vi "uService GUI.vi"(8 "error in (no error)":errorcluster, 11 "uService Template in":refnum<class "Scheduler.lvclass">) -> (3 "uService Template out":refnum<class "Scheduler.lvclass">)   [LabVIEW 2020, in "Scheduler.lvlib" / "Scheduler.lvclass"]
uses:
  Scheduler.lvclass
  C:/LabVIEW Code/CIRCUS/TALOS/TALOS_PPL.lvlibp/Father of all uServices/Father of all uServices/Father of all uServices.lvclass
  Run Utilities/Sequence of SBlocks/Sequence of SBlcoks - GUI.ctl
  Run Utilities/Schedule Block/Schedule Block - simplified GUI.ctl
  Run Utilities/TypeDefs/Synchronize FPGA Cluster.ctl
  Append Options.ctl
  Scheduler Consumer Case Selector.ctl
  Selection.ctl
  TALOS/TALOS_PPL.lvlibp/Father of all uServices/Father of all uServices/Father of all uServices.lvclass
  Scheduler.lvclass/Scheduler.ctl
  C:/LabVIEW Code/CIRCUS/TALOS/TALOS_PPL.lvlibp/Ancestor/Ancestor/Ancestor.lvclass
  C:/LabVIEW Code/CIRCUS/TALOS/Actor Framework.lvlibp/1abvi3w/vi.lib/ActorFramework/Actor/Actor.lvclass
  C:/LabVIEW Code/CIRCUS/CIRCUS uServices et al/Scheduler/Scheduler.lvclass
  Run Utilities/Sequence of SBlocks/Sequence of SBlocks.lvclass
  Run Utilities/Run Utilities.lvlib
  Run Utilities/Schedule Block/Schedule Block.lvclass
panel:
  in  "Append":T1
  in  "SB Buttons":T2
  in  "Add RUN":bool
  out "Sync. mask":T3[](array[typedef])
  in  "Parallel":bool
  in  "Reload parameters":bool
  in  "Array of Sequences":T4[](array[typedef])
  in  "Science":bool
  in  "Save":bool
  in  "Load":bool
  in  "Reset":bool
  in  "stop Scheduler":bool
  # "SCHEDULER"
  # "Schedule block manipulation"
  # "Multi FPGA Operation"
  # "Sync. mask"
  # "Estimated time of execution"
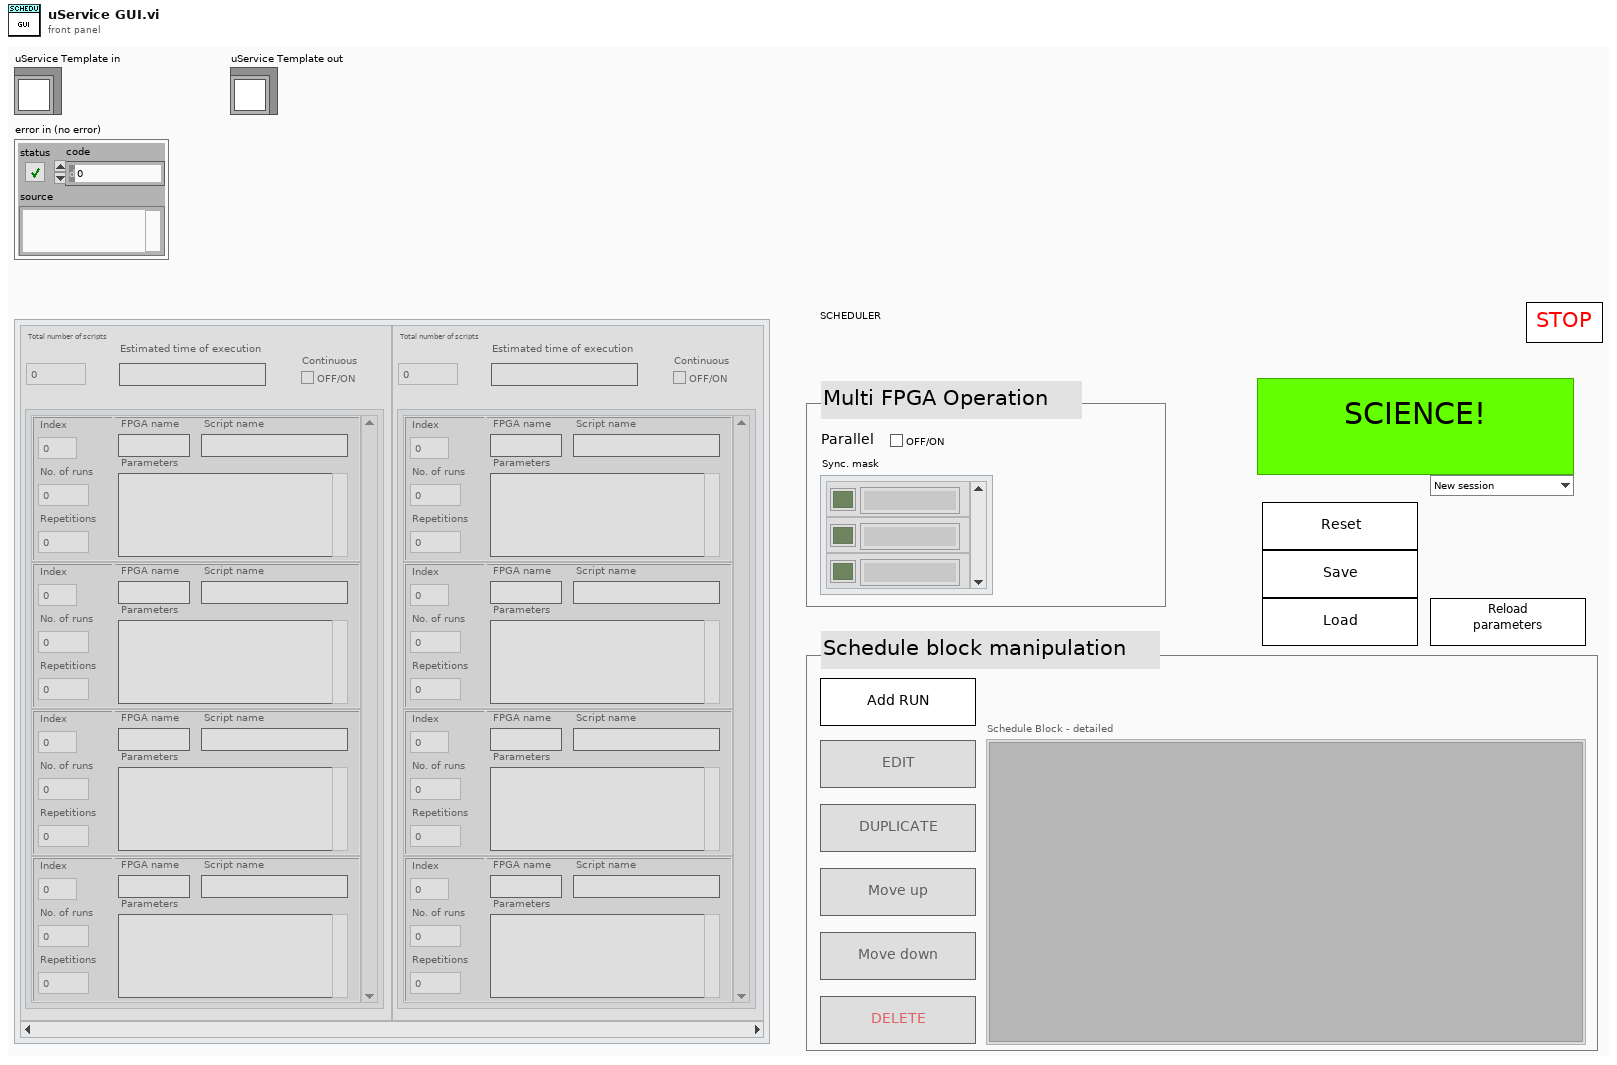
[diagram p1: front panel]
types:
  T1 = typedef "Scheduler.lvlib/Scheduler.lvclass/Append Options.ctl" = enum16{"New session", "Append to bottom", "Append to top"}
  T2 = cluster{"Move up SB":bool, "Move down SB":bool, "DELETE_SB":bool, "DUPLICATE_SB":bool, "EDIT_SB":bool}
  T3 = typedef "Run Utilities.lvlib/Synchronize FPGA Cluster.ctl" = cluster{"Status":bool, "FPGA Name":string}
  T4 = typedef "Run Utilities.lvlib/Sequence of SBlocks.lvclass/Sequence of SBlcoks - GUI.ctl" = cluster{"Total number of scripts":i32, "Time":string, "Sequence of SBlocks":T5[], "Continuous":bool}
  T5 = typedef "Run Utilities.lvlib/Schedule Block.lvclass/Schedule Block - simplified GUI.ctl" = cluster{"Bcg Color":u32, "Index":i32, "No. of runs":i32, "Script name":string, "FPGA name":string, "Parameters":string, "Repetitions":i32}
  T6 = enum16{"New session", "Append to bottom", "Append to top"}
  T7 = typedef "Scheduler.lvlib/Scheduler.lvclass/Scheduler Consumer Case Selector.ctl" = enum16{"Add SBlock", "Update GUI", "Move SBlock", "Select SBlock", "Update Cont.", "Load", "Save", "Reset", "Send to Tamer", "Edit SBlock", "Duplicate SBlock", "Delete SBlock", "Update SBlock", "Init", "Split/Combine Schedules", "Reschedule", "Load Parameters"}
  T8 = typedef "Scheduler.lvlib/Scheduler.lvclass/Selection.ctl" = cluster{"Row":i32, "Column":i32}
  T9 = typedef "TALOS.lvlib/Run Utilities.lvlib/Synchronize Kasli Cluster.ctl" = cluster{"Status":bool, "FPGA Name":string}
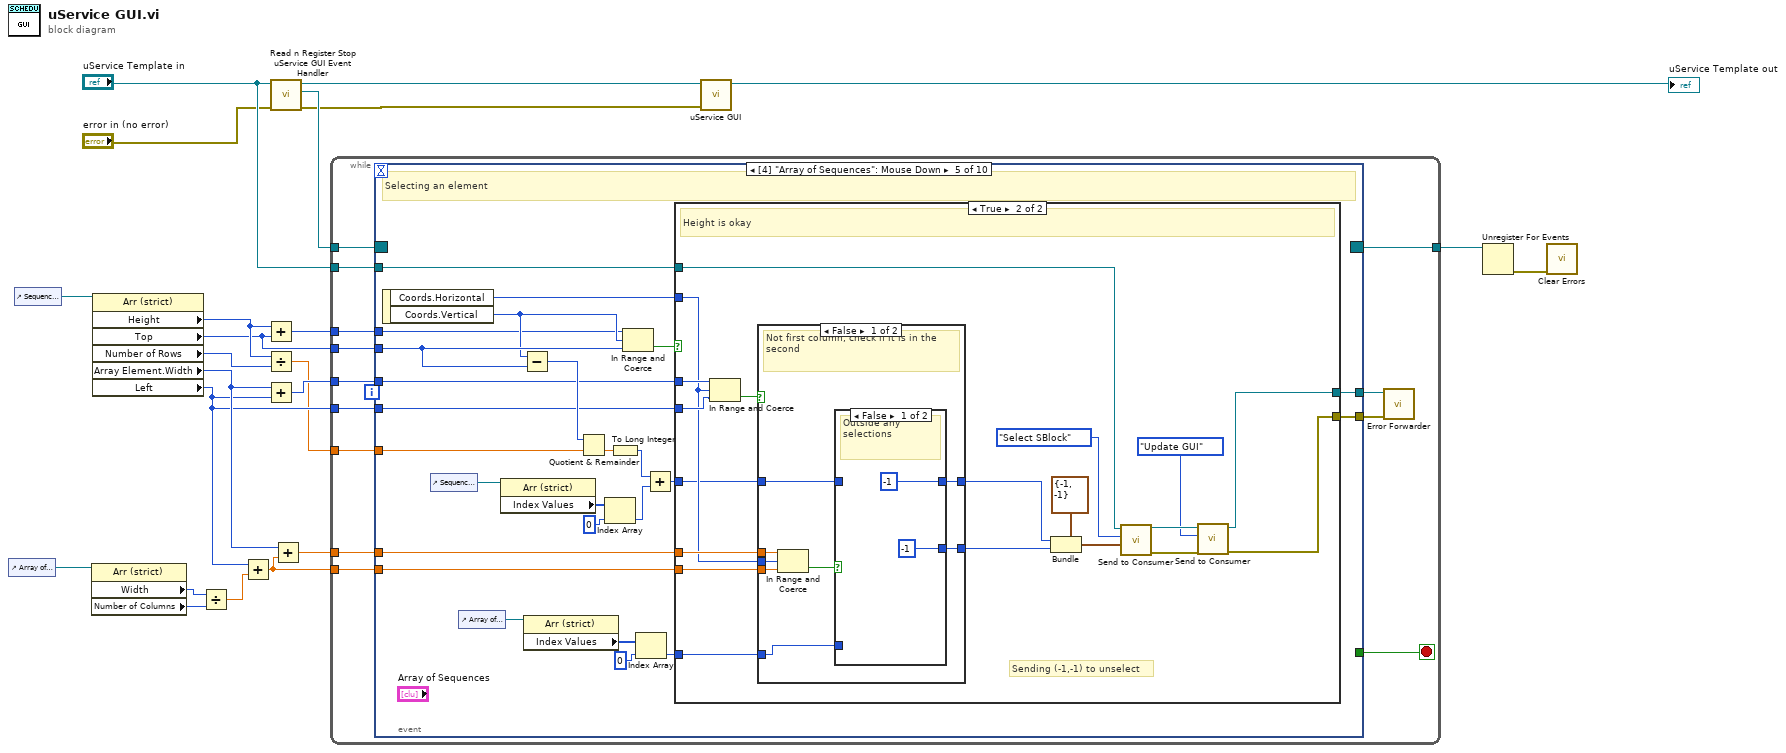
[diagram p0: block diagram]
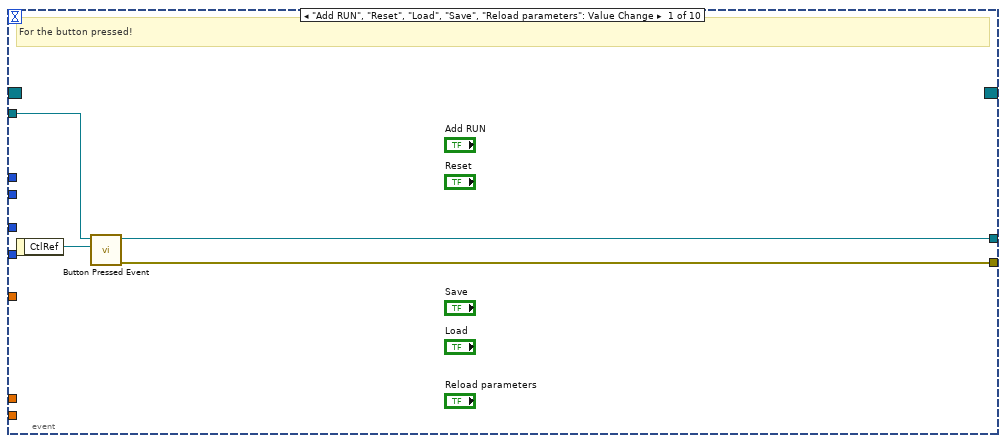
[diagram p2: hidden frame]
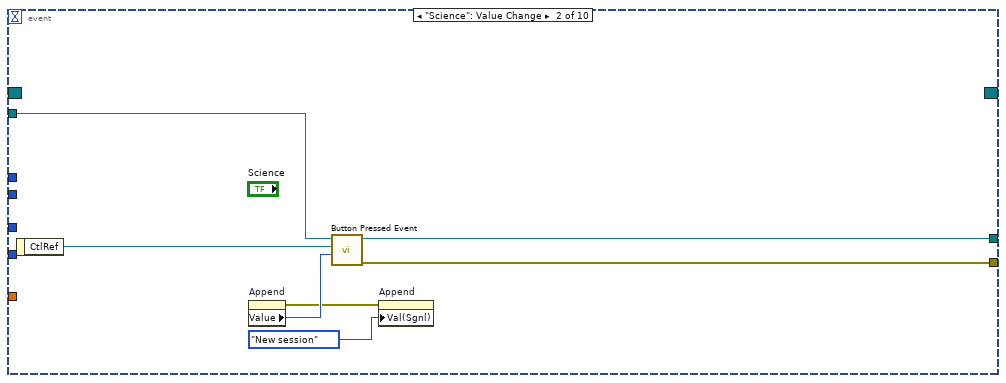
[diagram p3: hidden frame]
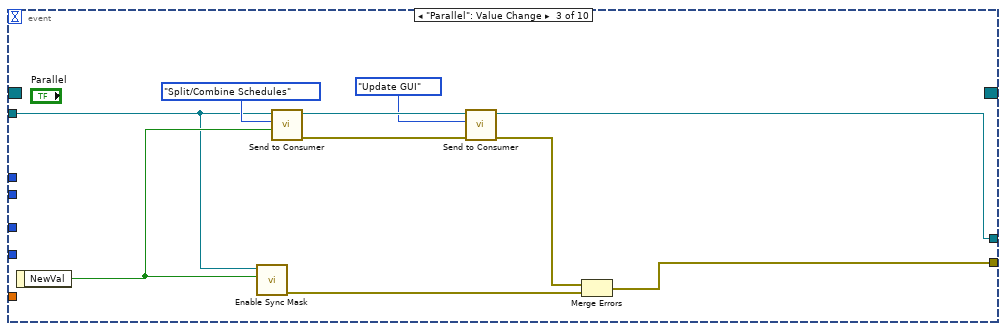
[diagram p4: hidden frame]
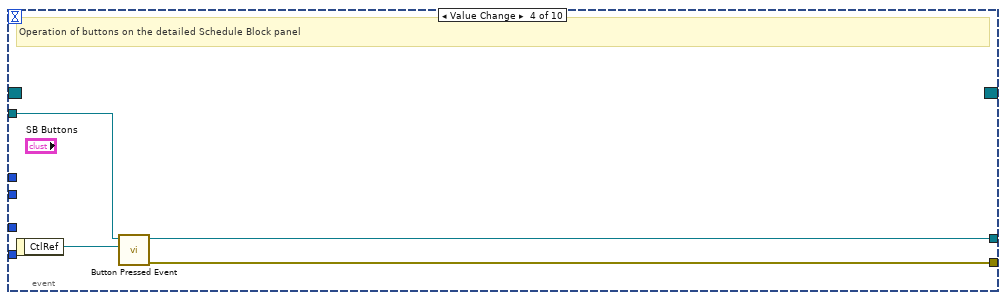
[diagram p5: hidden frame]
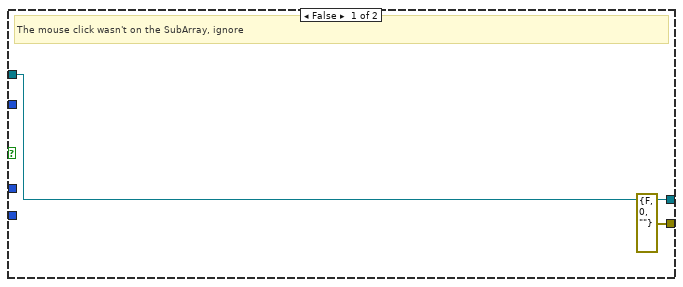
[diagram p6: hidden frame]
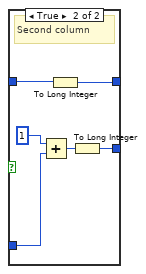
[diagram p7: hidden frame]
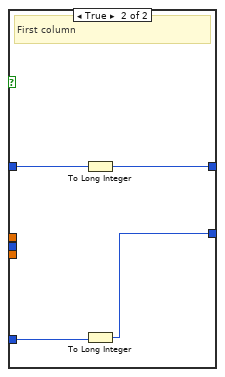
[diagram p8: hidden frame]
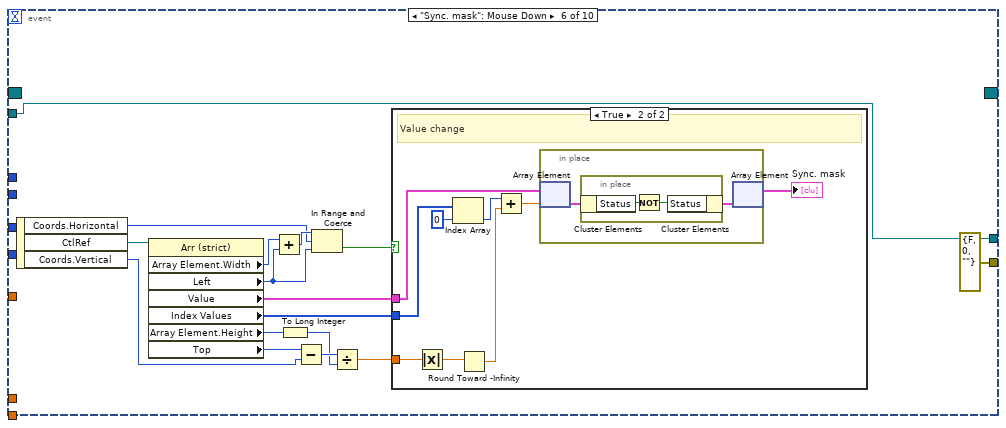
[diagram p9: hidden frame]
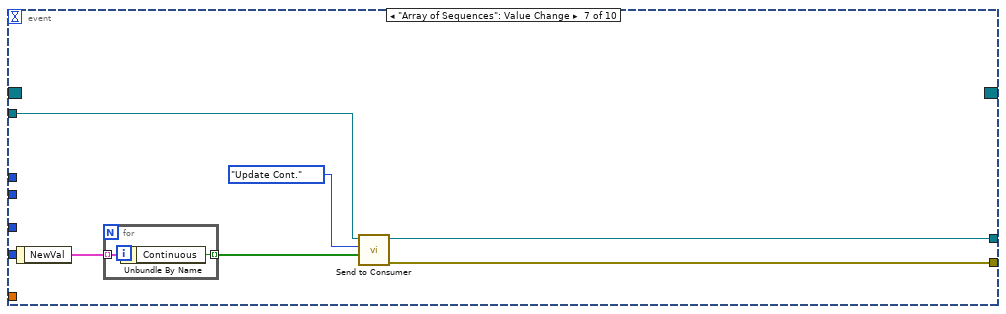
[diagram p11: hidden frame]
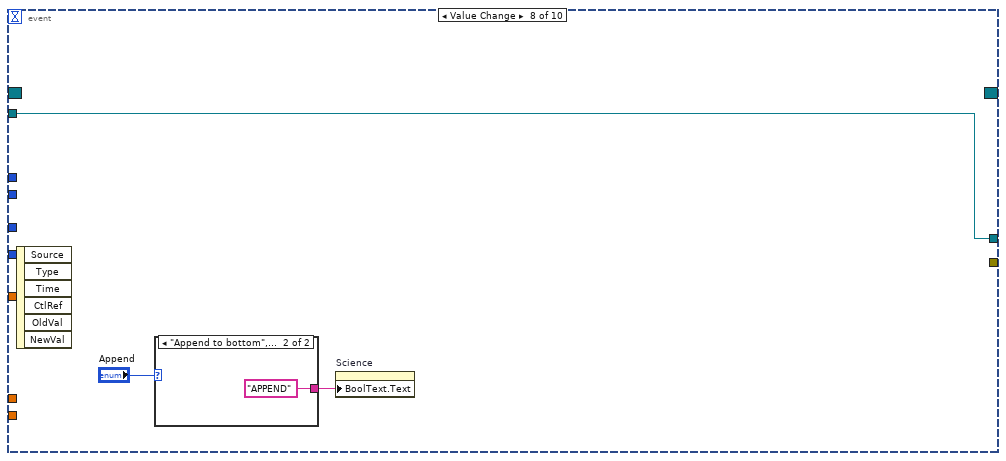
[diagram p12: hidden frame]
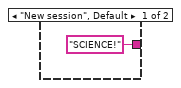
[diagram p13: hidden frame]
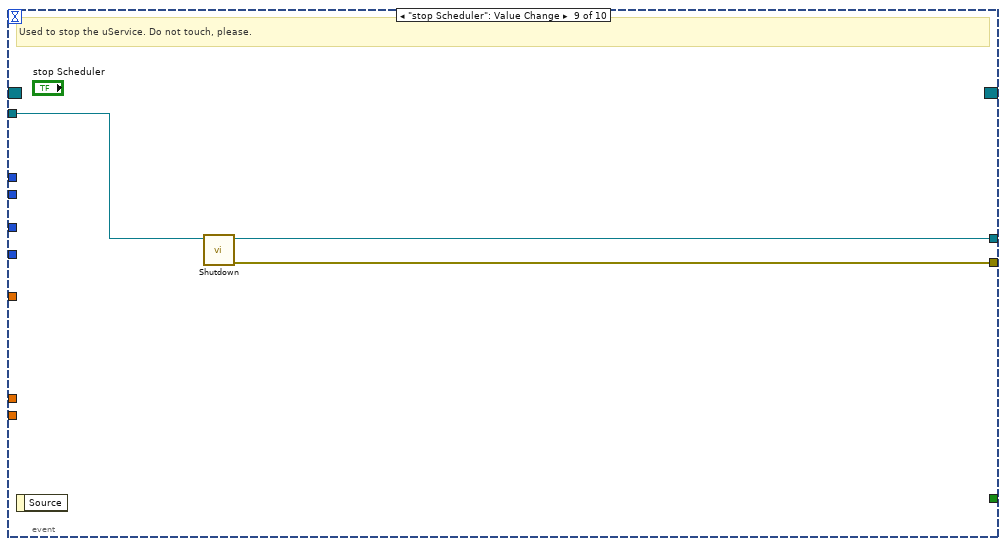
[diagram p14: hidden frame]
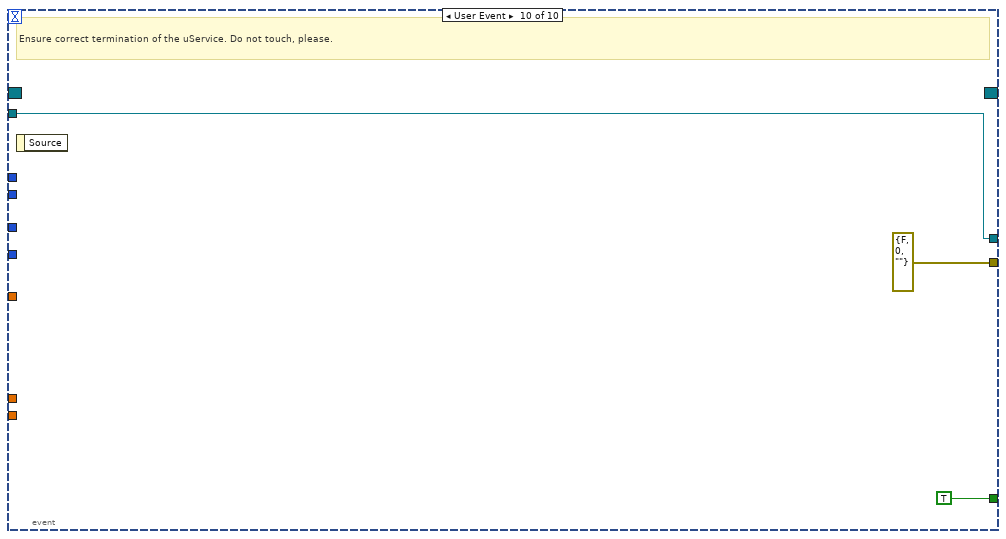
[diagram p15: hidden frame]
diagram:
  n1 = control-ref of="Array of Sequences"() -> (w5:refnum<vi>)
  n2 = control-ref of="Sequence of SBlocks"() -> (w4:refnum<vi>)
  n3 = property class="Arr (strict)"(reference=w5) -> ("Width"=w17:u32, "Number of Columns"=w2:u32)  [unwired: 1 in, 2 out]
  n4 = property class="Arr (strict)"(reference=w4) -> ("Height"=w16:u32, "Top"=w11:i32, "Number of Rows"=w15:u32, "Array Element.Width"=w13:u32, "Left"=w9:i32)  [unwired: 1 in, 2 out]
  n5 = Divide(x=w17, y=w2) -> (x/y=w14:dbl)
  n6 = Add(x=w9, y=w14) -> (x+y=w6:dbl)
  n7 = Add(x=w16, y=w11) -> (x+y=w12:u32)
  n8 = Divide(x=w16, y=w15) -> (x/y=w8:dbl)
  n9 = Add(x=w13, y=w9) -> (x+y=w10:u32)
  n10 = call-dynamic "Read n Register Stop uService GUI Event Handler .vi"("error in (no error)"="error in (no error)", "uService Template in"="uService Template in") -> ("error out"=w3:errorcluster, "Stop uService GUI Event Ref"=w18:refnum<event-registration>, "uService Template out"=w19:refnum<class "Scheduler.lvclass">)  [unwired: 7 in]
  n11 = Add(x=w13, y=w6) -> (x+y=w7:dbl)
  n12 = while {
    tunnel: [w36] -> w20
    tunnel: w18 -> [w34]
    tunnel: "uService Template in" -> [w33]
    tunnel: w12 -> [w32]
    tunnel: w11 -> [w31]
    tunnel: w10 -> [w30]
    tunnel: w9 -> [w29]
    tunnel: w8 -> [w28]
    tunnel: w7 -> [w27]
    tunnel: w6 -> [w26]
    stop <- w35 stop-if-true
    n13 = event shown="[4] \"Array of Sequences\": Mouse Down" {
      selector: w34 -> [_ _ _ _ _ _ _ _ _ _]
      dyn-events: [_ _ _ _ _ _ _ _ _ _] -> w36
      timeout: _ -> [_ _ _ _ _ _ _ _ _ _]
      tunnel: [_ _ _ _ _ _ _ _ _ TRUE] -> w35
      tunnel: w33 -> [w40 w47 w52 w60 w68 w129 w161 w167 w172 w174]
      tunnel: w32 -> [_ _ _ _ w64 _ _ _ _ _]
      tunnel: w31 -> [_ _ _ _ w75 _ _ _ _ _]
      tunnel: w30 -> [_ _ _ _ w74 _ _ _ _ _]
      tunnel: w29 -> [_ _ _ _ w73 _ _ _ _ _]
      tunnel: w28 -> [_ _ _ _ w72 _ _ _ _ _]
      tunnel: w27 -> [_ _ _ _ w71 _ _ _ _ _]
      tunnel: w26 -> [_ _ _ _ w65 _ _ _ _ _]
      tunnel: [w38 w46 w48 w59 w63 w129 w158 w167 w171 w174] -> w25
      tunnel: [w37 w45 w49 w58 w62 errorcluster {"status"=FALSE, "code"=0, "source"=""} ("error out") w157 _ w170 errorcluster {"status"=FALSE, "code"=0, "source"=""} ("error out")] -> w24
      event "Add RUN", "Reset", "Load", "Save", "Reload parameters": Value Change {
        # "For the button pressed!"
        n14 = event-data() -> ("CtlRef"=w39:refnum<vi>)  [unwired: 1 in]
        n15 = call-dynamic "Button Pressed Event.vi"("CtlRef"=w39, "uService Template in"=w40) -> ("error out"=w37:errorcluster, "uService Template out"=w38:refnum<class "Scheduler.lvclass">)  [unwired: 8 in]
      }
      event "Science": Value Change {
        n16 = event-data() -> ("CtlRef"=w44:refnum<vi>)  [unwired: 1 in]
        n17 = property on="Append" class="Enum (strict)"() -> (error out=w41:errorcluster, "Value"=w43:T1)  [unwired: 2 in, 1 out]
        n18 = call-dynamic "Button Pressed Event.vi"("Data"=w43, "CtlRef"=w44, "uService Template in"=w47) -> ("error out"=w45:errorcluster, "uService Template out"=w46:refnum<class "Scheduler.lvclass">)  [unwired: 7 in]
        n19 = property on="Append" class="Enum (strict)"(error in=w41, "Val(Sgnl)"=T6."New session" ("Append")) -> ()  [unwired: 1 in, 2 out]
      }
      event "Parallel": Value Change {
        n20 = event-data() -> ("NewVal"=w53:bool)  [unwired: 1 in]
        n21 = call-dynamic "Enable Sync Mask.vi"("Enable"=w53, "Scheduler in"=w52) -> ("error out"=w50:errorcluster)  [unwired: 8 in, 1 out]
        n22 = call "Send to Consumer.vi"("Data"=w53, "Case ID"=Scheduler_Consumer_Case_Selector."Split/Combine Schedules" ("Shifter Panel Consumer Case Selector"), "uService Template in"=w52) -> ("error out"=w54:errorcluster, "uService Template out"=w57:refnum<class "Scheduler.lvclass">)  [unwired: 7 in]
        n23 = call "Send to Consumer.vi"("error in (no error)"=w54, "Case ID"=Scheduler_Consumer_Case_Selector."Update GUI" ("Shifter Panel Consumer Case Selector"), "uService Template in"=w57) -> ("error out"=w51:errorcluster, "uService Template out"=w48:refnum<class "Scheduler.lvclass">)  [unwired: 7 in]
        n24 = Merge Errors(w51, w50) -> (w49:errorcluster)
      }
      event "SB Buttons.Move up SB", "SB Buttons.Move down SB", "SB Buttons.DELETE_SB", "SB Buttons.DUPLICATE_SB", "SB Buttons.EDIT_SB": Value Change {
        # "Operation of buttons on the detailed Schedule Block panel"
        n25 = event-data() -> ("CtlRef"=w61:refnum<vi>)  [unwired: 1 in]
        n26 = call-dynamic "Button Pressed Event.vi"("CtlRef"=w61, "uService Template in"=w60) -> ("error out"=w58:errorcluster, "uService Template out"=w59:refnum<class "Scheduler.lvclass">)  [unwired: 8 in]
      }
      event "Array of Sequences": Mouse Down {
        # "Selecting an element"
        n27 = event-data() -> ("Coords.Horizontal"=w70:i32, "Coords.Vertical"=w69:i32)  [unwired: 1 in]
        n28 = control-ref of="Sequence of SBlocks"() -> (w67:refnum<vi>)
        n29 = control-ref of="Array of Sequences"() -> (w66:refnum<vi>)
        n30 = property class="Arr (strict)"(reference=w67) -> ("Index Values"=w80:u32[])  [unwired: 1 in, 2 out]
        n31 = Subtract(x=w69, y=w75) -> (x-y=w82:i32)
        n32 = property class="Arr (strict)"(reference=w66) -> ("Index Values"=w85:u32[])  [unwired: 1 in, 2 out]
        n33 = Quotient & Remainder(x=w82, y=w72) -> (floor(x/y)=w81:dbl)  [unwired: 1 out]
        n34 = Index Array(array=w80, index=0) -> (element=w77:u32)
        n35 = To Long Integer(number=w81) -> (32bit integer=w79:i32)
        n36 = In Range and Coerce(upper limit=w64, x=w69, lower limit=w75) -> (In Range?=w86:bool)  [unwired: 1 out]
        n37 = Index Array(array=w85, index=0) -> (element=w83:u32)
        n38 = Add(x=w79, y=w77) -> (x+y=w76:u32)
        n39 = case shown="True" w86 {
          tunnel: w74 -> [_ w107]
          tunnel: w73 -> [_ w106]
          tunnel: w70 -> [_ w102]
          tunnel: w71 -> [_ w104]
          tunnel: w65 -> [_ w103]
          tunnel: w83 -> [_ w101]
          tunnel: w76 -> [_ w100]
          tunnel: w68 -> [w88 w99]
          tunnel: [w88 w89] -> w63
          tunnel: [errorcluster {"status"=FALSE, "code"=0, "source"=""} ("error out") w90] -> w62
          frame False {
            # "The mouse click wasn't on the SubArray, ignore"
          }
          frame True {
            # "Sending (-1,-1) to unselect"
            # "Height is okay"
            n40 = In Range and Coerce(upper limit=w107, x=w102, lower limit=w106) -> (In Range?=w105:bool)  [unwired: 1 out]
            n41 = case shown="False" w105 {
              tunnel: w104 -> [w115 _]
              tunnel: w103 -> [w114 _]
              tunnel: w102 -> [w113 _]
              tunnel: w101 -> [w111 w125]
              tunnel: w100 -> [w110 w127]
              tunnel: [w109 w126] -> w98
              tunnel: [w108 w124] -> w97
              frame False {
                # "Not first column, check if it is in the second"
                n42 = In Range and Coerce(upper limit=w115, x=w113, lower limit=w114) -> (In Range?=w112:bool)  [unwired: 1 out]
                n43 = case shown="False" w112 {
                  tunnel: w111 -> [_ w122]
                  tunnel: w110 -> [_ w121]
                  tunnel: [-1 w120] -> w109
                  tunnel: [-1 w118] -> w108
                  frame False {
                    # "Outside any selections"
                  }
                  frame True {
                    # "Second column"
                    n44 = Add(x=1, y=w122) -> (x+y=w119:u32)
                    n45 = To Long Integer(number=w121) -> (32bit integer=w120:i32)
                    n46 = To Long Integer(number=w119) -> (32bit integer=w118:i32)
                  }
                }
              }
              frame True {
                # "First column"
                n47 = To Long Integer(number=w127) -> (32bit integer=w126:i32)
                n48 = To Long Integer(number=w125) -> (32bit integer=w124:i32)
              }
            }
            n49 = Bundle(cluster=T8 {"Row"=-1, "Column"=-1} ("Selection"), "Row"=w98, "Column"=w97) -> (w96:T8)
            n50 = call "Send to Consumer.vi"("Data"=w96, "Case ID"=Scheduler_Consumer_Case_Selector."Select SBlock" ("Shifter Panel Consumer Case Selector"), "uService Template in"=w99) -> ("error out"=w94:errorcluster, "uService Template out"=w92:refnum<class "Scheduler.lvclass">)  [unwired: 7 in]
            n51 = call "Send to Consumer.vi"("error in (no error)"=w94, "Case ID"=Scheduler_Consumer_Case_Selector."Update GUI" ("Shifter Panel Consumer Case Selector"), "uService Template in"=w92) -> ("error out"=w90:errorcluster, "uService Template out"=w89:refnum<class "Scheduler.lvclass">)  [unwired: 7 in]
          }
        }
      }
      event "Sync. mask": Mouse Down {
        n52 = event-data() -> ("Coords.Horizontal"=w139:i32, "CtlRef"=w143:refnum<vi>, "Coords.Vertical"=w133:i32)  [unwired: 1 in]
        n53 = property class="Arr (strict)"(reference=w143) -> ("Array Element.Width"=w141:u32, "Left"=w140:i32, "Value"=w136:T9[], "Index Values"=w135:u32[], "Array Element.Height"=w137:u32, "Top"=w134:i32)  [unwired: 1 in, 2 out]
        n54 = Add(x=w141, y=w140) -> (x+y=w142:u32)
        n55 = To Long Integer(number=w137) -> (32bit integer=w131:i32)
        n56 = Subtract(x=w134, y=w133) -> (x-y=w132:i32)
        n57 = In Range and Coerce(upper limit=w142, x=w139, lower limit=w140) -> (In Range?=w138:bool)  [unwired: 1 out]
        n58 = Divide(x=w132, y=w131) -> (x/y=w130:dbl)
        n59 = case shown="True" w138 {
          tunnel: w136 -> [_ w148]
          tunnel: w135 -> [_ w150]
          tunnel: w130 -> [_ w152]
          frame False {
            # "This is just scrolling"
          }
          frame True {
            # "Value change"
            n60 = Absolute Value(x=w152) -> (abs(x)=w151:dbl)
            n61 = Index Array(array=w150, index=0) -> (element=w146:u32)
            n62 = Round Toward -Infinity(1:w151) -> (0:w147:dbl)
            n63 = Add(x=w146, y=w147) -> (x+y=w145:dbl)
            n64 = in-place {
              n65 = in-place-array #1(w148, w145) -> (w154:T9)
              n66 = in-place {
                n67 = in-place-cluster #2(w154) -> ("Status"=w156:bool)
                n68 = Not(x=w156) -> (.not. x?=w155:bool)
                n69 = in-place-cluster #2("Status"=w155) -> (w153:T9)
              }
              n70 = in-place-array #1(w153) -> (→"Sync. mask":T9[])  [unwired: 1 out]
            }
          }
        }
      }
      event "Array of Sequences": Value Change {
        n71 = event-data() -> ("NewVal"=w162:T4[])  [unwired: 1 in]
        n72 = for {
          tunnel: w162 -> [w164] mode=indexing
          tunnel: [w163] -> w160 mode=indexing
          n73 = Unbundle By Name(w164) -> ("Continuous"=w163:bool)
        }
        n74 = call "Send to Consumer.vi"("Data"=w160, "Case ID"=Scheduler_Consumer_Case_Selector."Update Cont." ("Shifter Panel Consumer Case Selector"), "uService Template in"=w161) -> ("error out"=w157:errorcluster, "uService Template out"=w158:refnum<class "Scheduler.lvclass">)  [unwired: 7 in]
      }
      event Value Change {
        n75 = event-data() -> ()  [unwired: 1 in, 6 out]
        n76 = case shown="\"Append to bottom\", \"Append to top\"" "Append" {
          tunnel: ["SCIENCE!" ("Boolean Text.Text") "APPEND" ("Boolean Text.Text")] -> w165
          frame "New session", Default {
          }
          frame "Append to bottom", "Append to top" {
          }
        }
        n77 = property on="Science" class="Bool"("BoolText.Text"=w165) -> ()  [unwired: 2 in, 2 out]
      }
      event "stop Scheduler": Value Change {
        # "Used to stop the uService. Do not touch, please."
        n78 = event-data() -> ()  [unwired: 1 in, 1 out]
        n79 = call "Shutdown.vi"("Father of all uServices in"=w172) -> ("error out"=w170:errorcluster, "Father of all uServices out"=w171:refnum<class "Scheduler.lvclass">)  [unwired: 9 in]
      }
      event User Event {
        # "Ensure correct termination of the uService. Do not touch, please."
        n80 = event-data() -> ()  [unwired: 1 in, 1 out]
      }
    }
    n81 = call "Error Forwarder.vi"("error in (no error)"=w24, "Father of all uServices in"=w25) -> ()  [unwired: 10 in]
  }
  n82 = call-parent "uService GUI.vi"("error in (no error)"=w3, "uService Template in"=w19) -> ("uService Template out"=→"uService Template out":refnum<class "Scheduler.lvclass">)  [unwired: 9 in]
  n83 = Unregister For Events(event registration refnum=w20) -> (error out=w1:errorcluster)  [unwired: 1 in]
  n84 = call <vilib>:"Clear Errors.vi"("error in (no error)"=w1) -> ()  [unwired: 5 in, 2 out]
